vi "Current_Setting_1_7_26_TC9_ramp_working.vi"() -> ()   [LabVIEW 2025]
uses:
  <vilib>/addons/zeromq/socket_type.ctl
  <vilib>/DAQmx/write.llb/DAQmx Write (Analog DBL 1Chan 1Samp).vi
  <vilib>/DAQmx/read.llb/DAQmx Read (Analog DBL 1Chan 1Samp).vi
  <vilib>/DAQmx/read.llb/DAQmx Read (Analog 1D DBL NChan 1Samp).vi
  <vilib>/DAQmx/create/channels.llb/DAQmx Create Channel (AI-Voltage-Basic).vi
  Trimming_Coil_Command.vi
  Trimming_Coil_Monitor.vi
  <vilib>/Waveform/DWDTOps.llb/DWDT Digital to Boolean Array.vi
  GV_TC1.vi
  <vilib>/DAQmx/miscellaneous.llb/DAQmx Fill In Error Info.vi
  <vilib>/DAQmx/create/channels.llb/DAQmx Create Channel (AO-Voltage-Basic).vi
  <vilib>/addons/zeromq/zmq_socket.lvclass
  <vilib>/addons/zeromq/zmq_context.lvclass
  <vilib>/addons/zeromq/zeromq.lvlib
  <resource>/objmgr/daqmx.rc
panel:
  out "Numeric":dbl
  in  "TC9_Set_Point":dbl
  in  "stop":bool
  out "TC1_Command":dbl
  out "Waveform Chart":dbl(graph)
  out "Sign*10":dbl
  in  "Error_TC9":dbl
  in  "Inc/Dec":dbl
  in  "RF":tag
  in  "Others":tag
  out "error out":errorcluster
  out "double precision float":dbl
  out "Source 1":dbl
  out "Source 2":dbl
  out "Source 3":dbl
  out "Source 4":dbl
  out "Source 5":dbl
  out "Source 6":dbl
  out "Source 7":dbl
  out "Source 8":dbl
  out "Source 9":dbl
  out "Source 10":dbl
  out "Source 11":dbl
  out "Source 12":dbl
  out "Source 13":dbl
  out "Source 14":dbl
  out "value":dbl[](array[numeric])
  out "subarray":dbl[](array[numeric])
  out "Boolean array":bool[](array[boolean])
  out "TC 1":dbl
  out "TC 2":dbl
  out "TC 3":dbl
  out "TC 4":dbl
  out "TC 5":dbl
  out "TC 6":dbl
  out "TC 7":dbl
  out "TC 8":dbl
  out "going to Device 9":dbl
  out "going to Device 10":dbl
  out "going to Device 11":dbl
  out "going to Device 12":dbl
  out "going to Device 13":dbl
  out "going to Device 14":dbl
  in  "Numerator":dbl
  in  "Denominator":dbl
  in  "Inc/Dec 2":dbl
  in  "Error_Stop":dbl
  in  "Boolean":bool
  out "Array":dbl[](array[numeric])
  out "max value":i16
  out "Array[0]":dbl
  out "Array 2":dbl[](array[numeric])
  in  "TP1":dbl
  in  "TP2":dbl
  in  "RF 2":dbl
  in  "Beam":dbl
  in  "Boolean 2":bool
  in  "Boolean 3":bool
  out "[0]":bool
  out "[1]":bool
  out "[2]":bool
  out "[3]":bool
  out "others":dbl[](array[numeric]) format="%0.2f"
  out "appended array":dbl[](array[numeric])
  out "x/y":dbl
  # "Beam I"
  # "ESD KV"
  # "ARC V"
  # "Filament C"
  # "Inside Iron"
  # "Outside Iron"
  # "ARC C"
  # "ESD mA"
  # "TC1"
  # "TC2"
  # "TC4"
  # "TC5"
  # "TC6"
  # "TC7"
  # "TC10"
  # "TC9"
  # "TP2"
  # "TP1"
  # "Filament V"
  # "Centering Beam"
  # "TC 12"
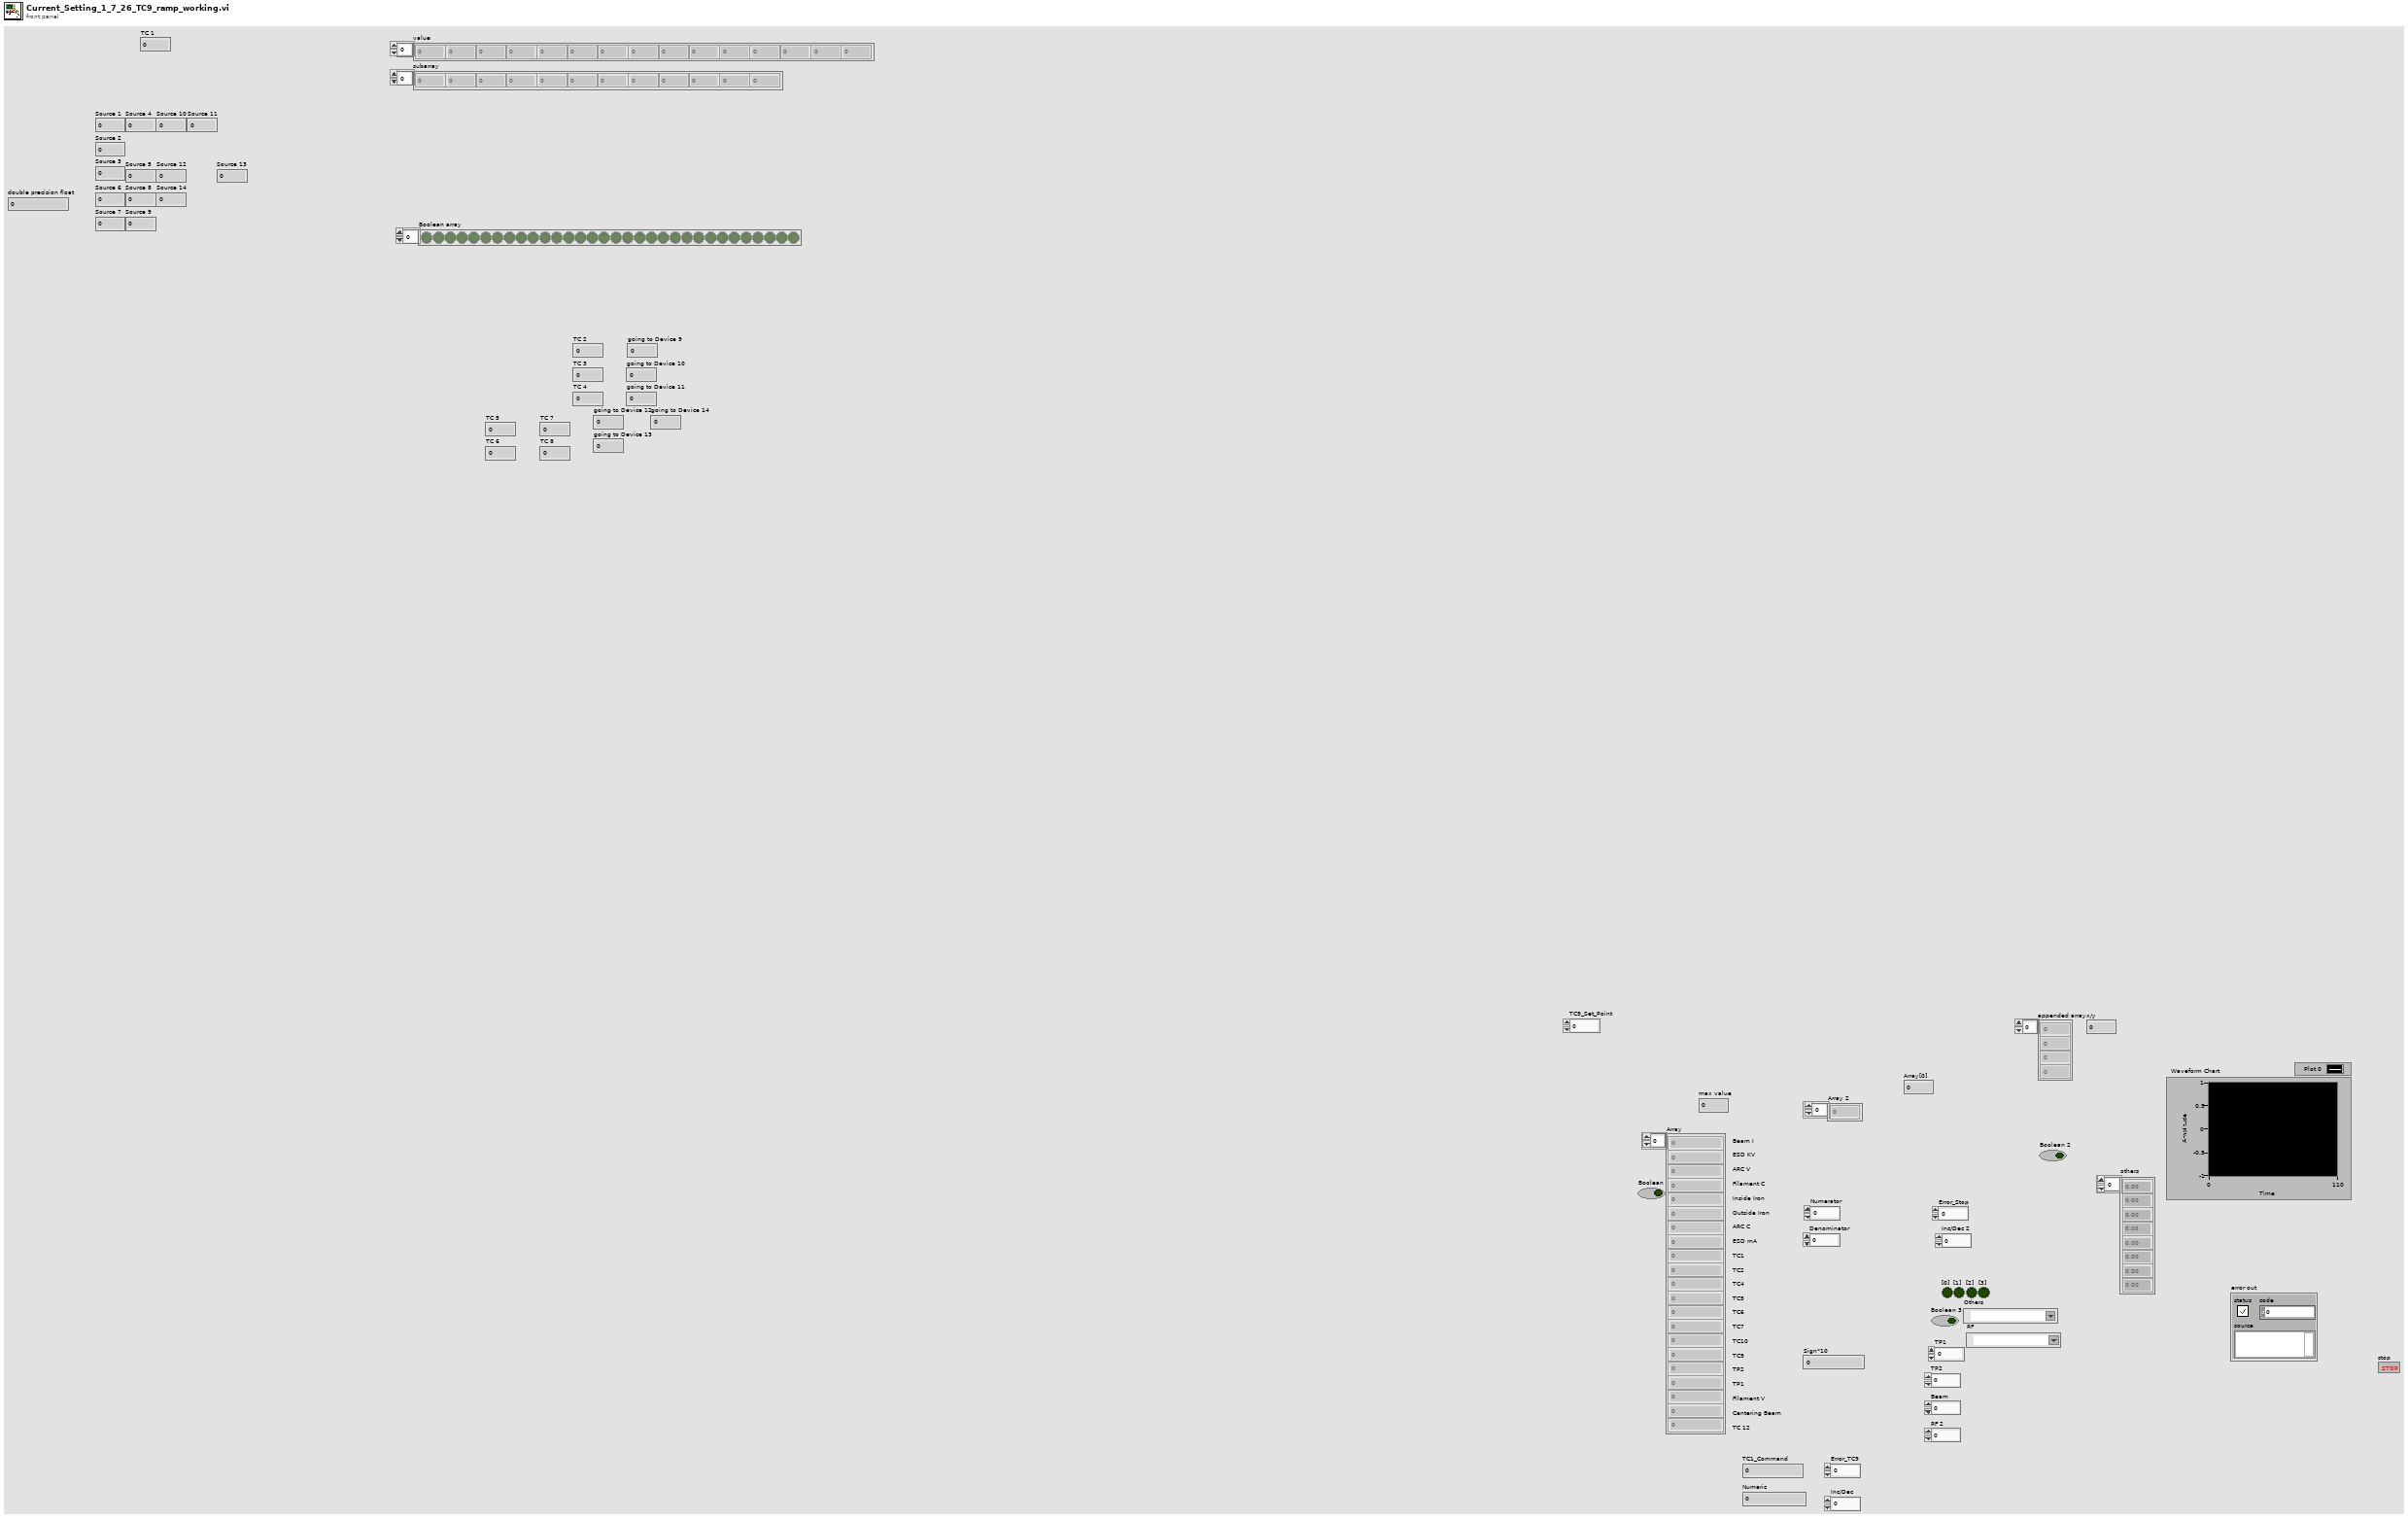
[diagram p1: front panel]
types:
  T1 = typedef "zeromq.lvlib/socket_type.ctl" = enum8{"ZMQ_PAIR", "ZMQ_PUB", "ZMQ_SUB", "ZMQ_REQ", "ZMQ_REP", "ZMQ_DEALER", "ZMQ_ROUTER", "ZMQ_PULL", "ZMQ_PUSH", "ZMQ_XPUB", "ZMQ_XSUB", "ZMQ_STREAM", "ZMQ_SERVER", "ZMQ_CLIENT", "ZMQ_RADIO", "ZMQ_DISH", "ZMQ_GATHER", "ZMQ_SCATTER", "ZMQ_DGRAM"}
  T2 = enum16{"big-endian, network order", "native, host order", "little-endian"}
  T3 = cluster{"TC1_Set_Point":dbl, "TC2_Set_Point":dbl, "TC3_Set_Point":dbl, "TC4_Set_Point":dbl, "TC5_Set_Point":dbl, "TC6_Set_Point":dbl, "TC7_Set_Point":dbl, "TC8_Set_Point":dbl, "TC9_Set_Point":dbl, "TC10_Set_Point":dbl, "TC11_Set_Point":dbl, "TC12_Set_Point":dbl}
  T4 = cluster{"[0]":bool, "[1]":bool, "[2]":bool, "[3]":bool, "[4]":bool, "[5]":bool, "[6]":bool, "[7]":bool, "[8]":bool}
  T5 = cluster{"[0]":dbl, "[1]":dbl, "[2]":dbl, "[3]":dbl, "[4]":dbl, "[5]":dbl, "[6]":dbl, "[7]":dbl}
  T6 = cluster{"Array[0]":dbl, "Array[1]":dbl, "Array[2]":dbl, "Array[3]":dbl, "Array[4]":dbl, "Array[5]":dbl, "Array[6]":dbl, "Array[7]":dbl}
  T7 = cluster{"[0]":digitalwaveform, "[1]":digitalwaveform, "[2]":digitalwaveform, "[3]":digitalwaveform, "[4]":digitalwaveform, "[5]":digitalwaveform, "[6]":digitalwaveform, "[7]":digitalwaveform, "[8]":digitalwaveform}
  T8 = cluster{"TC1_Readback":dbl, "TC2_Readback":dbl, "TC3_Readback":dbl, "TC4_Readback":dbl, "TC5_Readback":dbl, "TC6_Readback":dbl, "TC7_Readback":dbl, "TC8_Readback":dbl, "TC9_Readback":dbl, "TC10_Readback":dbl, "TC11_Readback":dbl, "TC12_Readback":dbl}
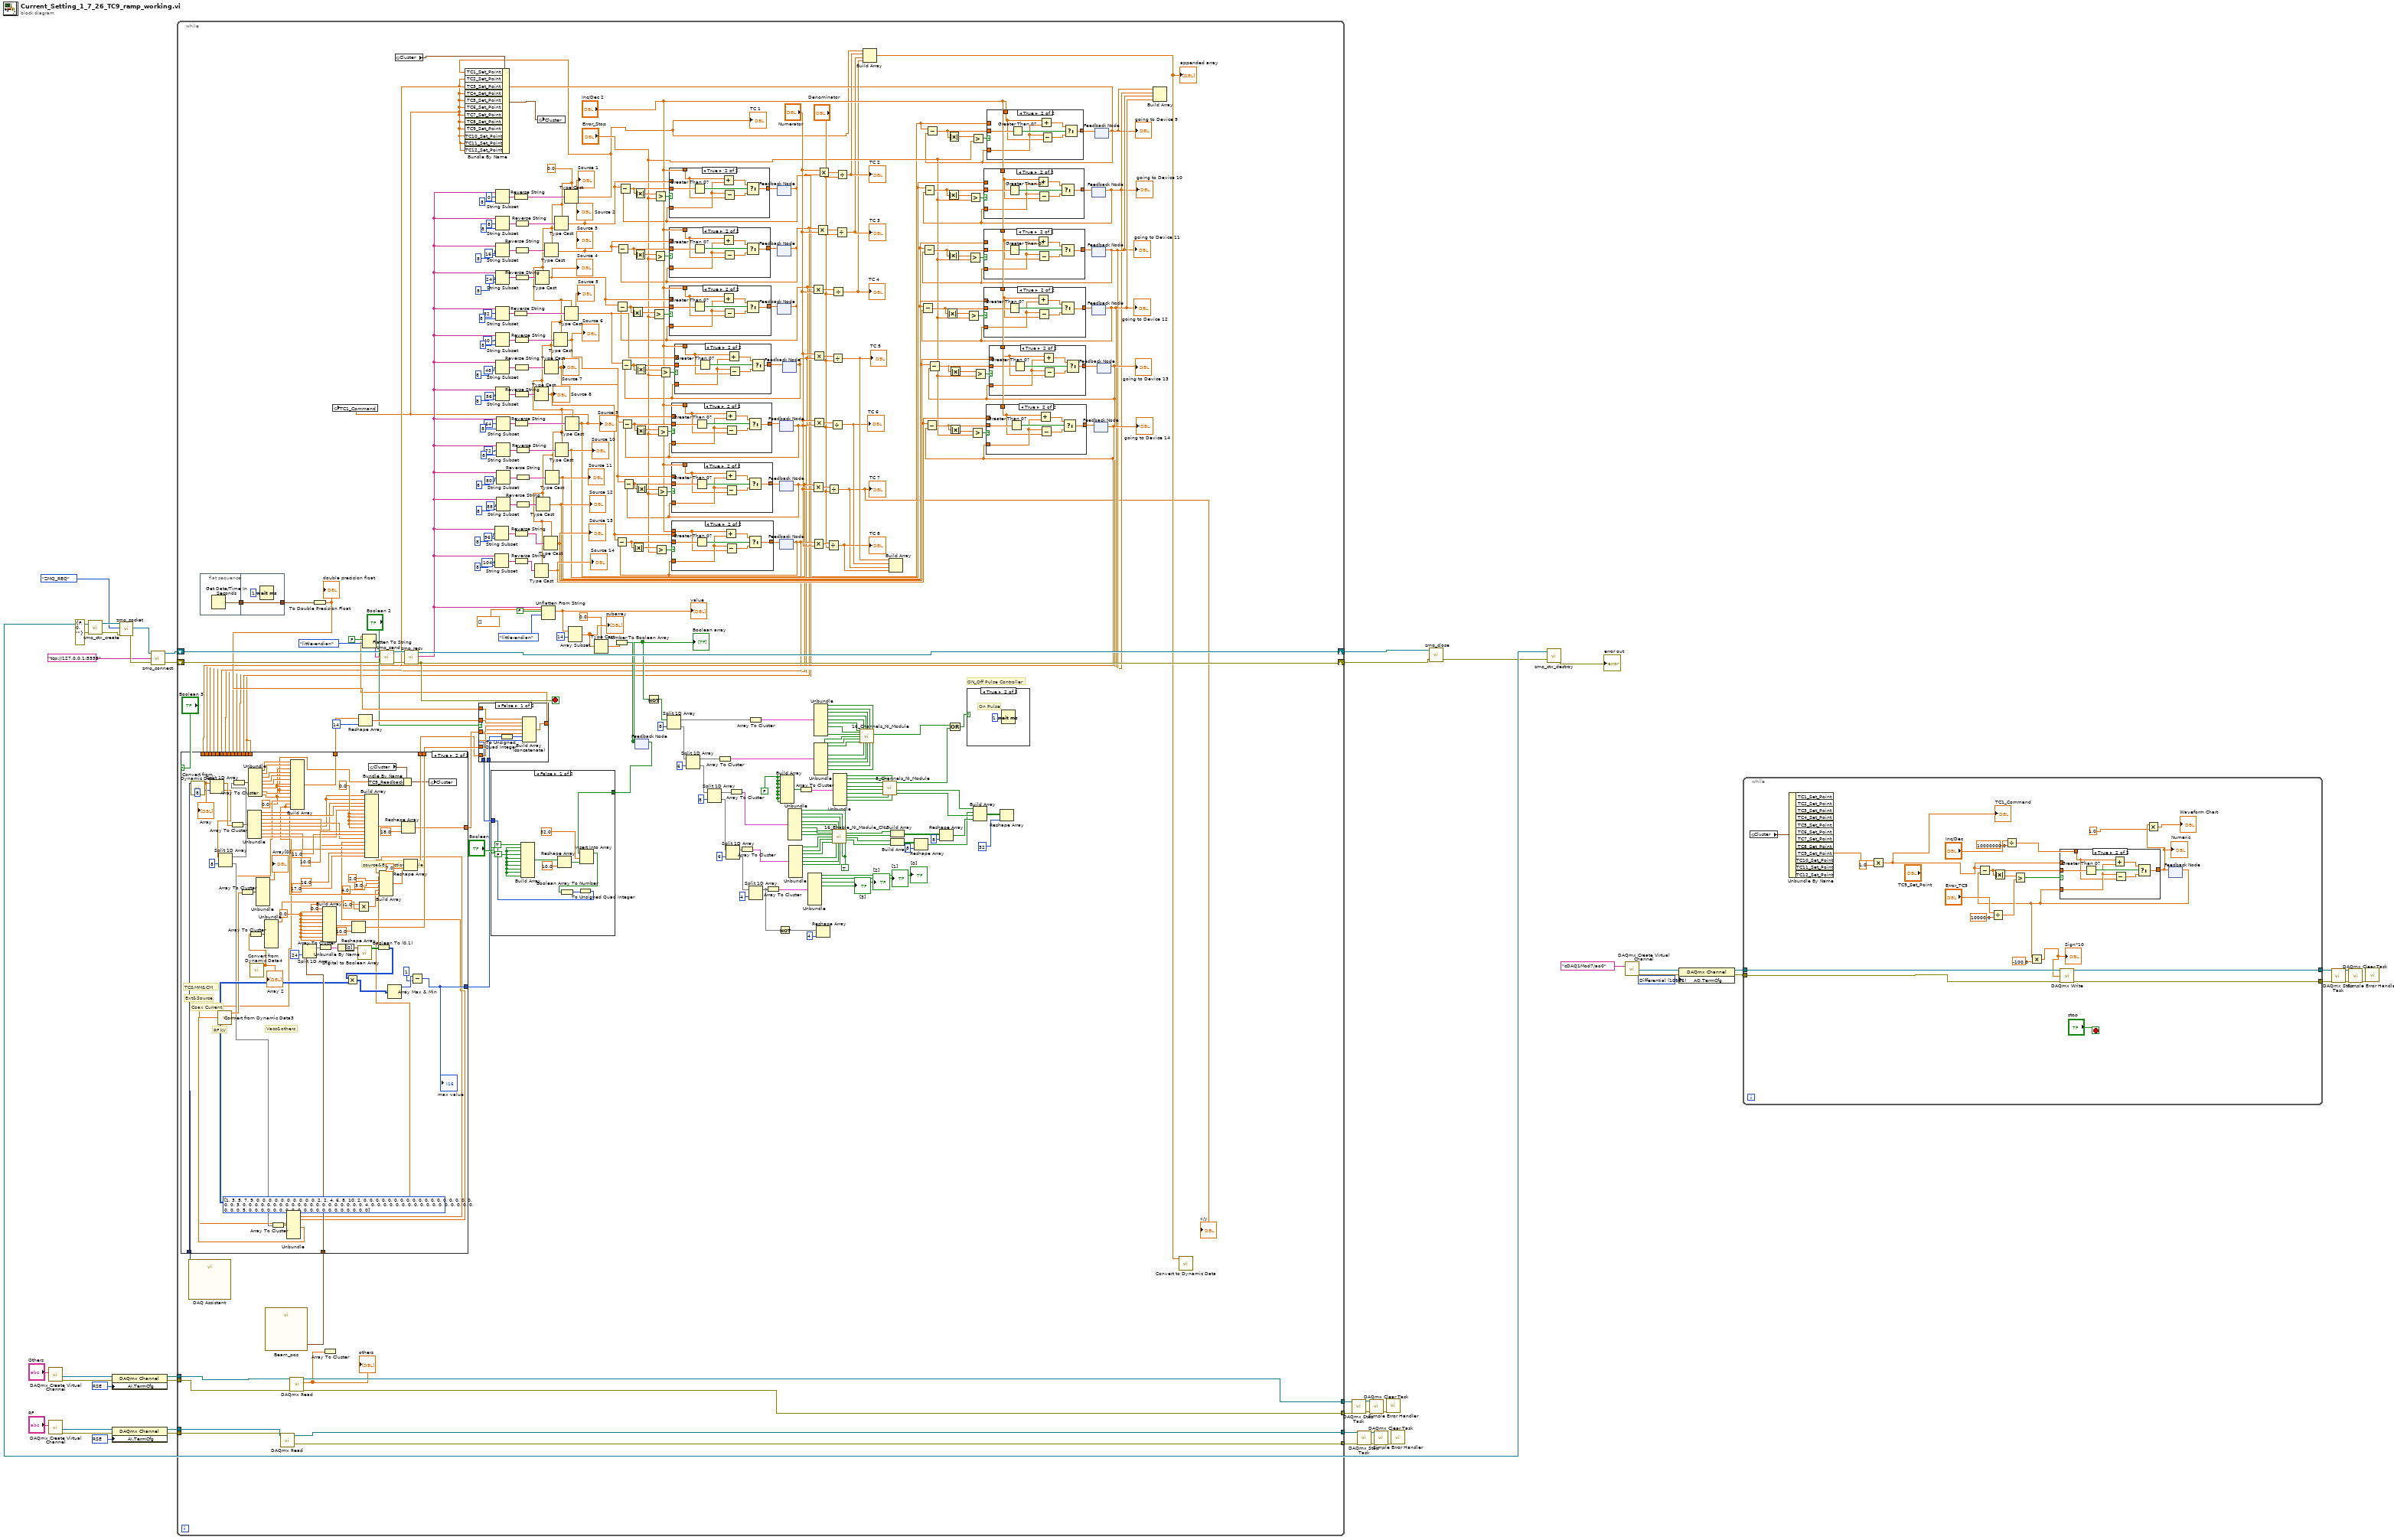
[diagram p0: block diagram]
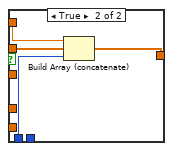
[diagram p3: hidden frame]
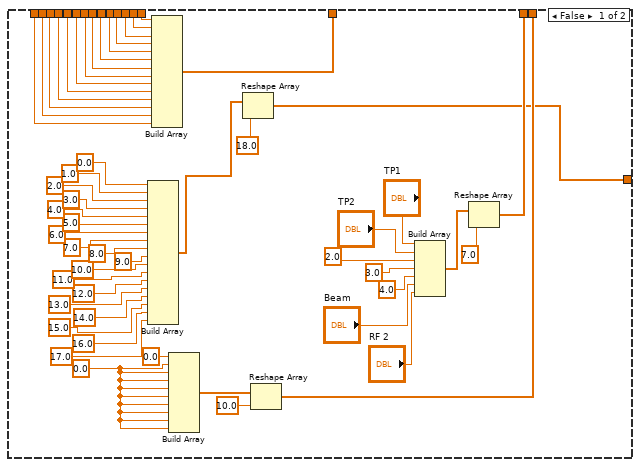
[diagram p4: hidden frame]
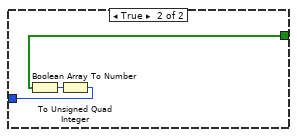
[diagram p5: hidden frame]
diagram:
  w8 = 10106 items=["RSE"=10083, "Differential"=10106, "Pseudodifferential"=12529] ("AO.TermCfg")
  w20 = 10083 items=["RSE"=10083, "Differential"=10106, "Pseudodifferential"=12529] ("AO.TermCfg")
  w31 = 10083 items=["RSE"=10083, "Differential"=10106, "Pseudodifferential"=12529] ("AO.TermCfg")
  n1 = call-poly <vilib>:"DAQmx Create Virtual Channel.vi"("physical channels"="Others") -> ("task out"=w32:refnum<k21>, "error out"=w33:errorcluster)  [unwired: 13 in]
  n2 = call-poly <vilib>:"DAQmx Create Virtual Channel.vi"("physical channels"="RF") -> ("task out"=w21:refnum<k21>, "error out"=w22:errorcluster)  [unwired: 13 in]
  n3 = call <vilib>:"zmq_ctx_create.vi"("error in"=errorcluster {"status"=FALSE, "code"=0, "source"=""}) -> ("error out"=w45:errorcluster, "context out"=w46:refnum<class "zmq_context.lvclass">)  [unwired: 3 in]
  n4 = property class="DAQmx Channel"(reference=w32, error in=w33, "AI.TermCfg"=w31) -> (reference out=w26:refnum<k21>, error out=w25:errorcluster)
  n5 = property class="DAQmx Channel"(reference=w21, error in=w22, "AI.TermCfg"=w20) -> (reference out=w18:refnum<k21>, error out=w17:errorcluster)
  n6 = call <vilib>:"zmq_socket.vi"("error in"=w45, "socket type"=socket_type."ZMQ_REQ", "context in"=w46) -> ("error out"=w43:errorcluster, "socket out"=w44:refnum<class "zmq_socket.lvclass">, "context out"=w38:refnum<class "zmq_context.lvclass">)  [unwired: 2 in]
  n7 = call <vilib>:"zmq_connect.vi"("error in"=w43, "endpoint"="tcp://127.0.0.1:5555", "socket in"=w44) -> ("error out"=w39:errorcluster, "socket out"=w40:refnum<class "zmq_socket.lvclass">)  [unwired: 1 in]
  n8 = while {
    shift-right: [w225] -> w35
    shift-left: w40 -> [w335]
    shift-right: [w224] -> w36
    shift-left: w39 -> [w334]
    tunnel: w26 -> [w82]
    tunnel: w25 -> [w81]
    tunnel: [w80] -> w24
    tunnel: [w79] -> w23
    tunnel: w18 -> [w78]
    tunnel: w17 -> [w77]
    tunnel: [w76] -> w13
    tunnel: [w75] -> w12
    stop <- w224 stop-if-true
    w115 = TRUE
    w118 = FALSE
    w52 = 0.0
    # "ON_Off Pulse Controller"
    n9 = call "DAQ Assistant"() -> ("data"=w57:dynamicdata)  [unwired: 16 in, 3 out]
    n10 = flat-sequence {
      tunnel: [w593] -> w330
      tunnel: [w595] -> w331
      tunnel: w330 -> [w595]
      frame #0 {
        n11 = Get Date/Time In Seconds() -> (seconds since 1Jan1904=w593:timestamp)
      }
      frame #1 {
        n12 = Wait (ms)(milliseconds to wait=u32 1) -> ()  [unwired: 1 out]
      }
    }
    n13 = call "Beam_pos"() -> ("data"=w58:digitalwaveform[])  [unwired: 16 in, 3 out]
    n14 = call-poly <vilib>:"DAQmx Read.vi"("task/channels in"=w78, "error in"=w77) -> ("task out"=w76:refnum<k21>, "error out"=w75:errorcluster)  [unwired: 11 in, 1 out]
    n15 = call-poly <vilib>:"DAQmx Read.vi"("task/channels in"=w82, "error in"=w81) -> ("task out"=w79:refnum<k21>, "data"=w74:dbl[], "error out"=w80:errorcluster)  [unwired: 11 in]
    "others" <- w74
    n16 = To Double Precision Float(number=w331) -> (double precision float=w102:dbl)
    "double precision float" <- w102
    n17 = Array To Cluster(array=w74) -> ()  [unwired: 1 out]
    n18 = global read "Trimming_Coil_Command.vi" "Cluster"() -> (w51:T3)
    n19 = feedback #1() -> (w105:bool[])  [unwired: 1 in]
    n20 = case shown="False" "Boolean" {
      tunnel: w105 -> [w480 w486]
      tunnel: [w477 w485] -> w103
      frame False {
        w483 = FALSE
        n21 = Build Array(TRUE, w483, w483, w483, w483, w483, w483, w483, w483, w483) -> (w482:bool[])
        n22 = Reshape Array(w482, 10.0) -> (w475:bool[])
        n23 = Insert Into Array(array=w480, index=32.0, new element=w475) -> (w478:bool[])
        n24 = Boolean Array To Number(Boolean array=w478) -> (number=w479:u32)
        n25 = To Unsigned Quad Integer(1:w479) -> (0:w477:u64)
      }
      frame True {
        n26 = Boolean Array To Number(Boolean array=w486) -> (number=w487:u32)
        n27 = To Unsigned Quad Integer(1:w487) -> (0:w485:u64)
      }
    }
    n28 = feedback #2() -> (w53:dbl)  [unwired: 1 in]
    n29 = feedback #3() -> (w62:dbl)  [unwired: 1 in]
    n30 = feedback #4() -> (w63:dbl)  [unwired: 1 in]
    n31 = feedback #5() -> (w65:dbl)  [unwired: 1 in]
    n32 = feedback #6() -> (w66:dbl)  [unwired: 1 in]
    n33 = feedback #7() -> (w67:dbl)  [unwired: 1 in]
    n34 = Build Array(w118, w118, w118, w118, w118, w118, w118, w118) -> (w116:bool[])
    n35 = feedback #8() -> (w64:dbl)  [unwired: 1 in]
    n36 = Array To Cluster(array=w116) -> (cluster=w117:T4)
    n37 = Multiply(x=w63, y="Numerator") -> (x*y=w219:dbl)
    n38 = Multiply(x=w66, y="Numerator") -> (x*y=w216:dbl)
    n39 = Multiply(x=w67, y="Numerator") -> (x*y=w215:dbl)
    n40 = Multiply(x="Numerator", y=w64) -> (x*y=w218:dbl)
    n41 = Multiply(x="Numerator", y=w65) -> (x*y=w217:dbl)
    n42 = Multiply(x=w62, y="Numerator") -> (x*y=w220:dbl)
    n43 = Multiply(x="Numerator", y=w53) -> (x*y=w221:dbl)
    n44 = Divide(x=w215, y="Denominator") -> (x/y=w106:dbl)
    "TC 8" <- w106
    n45 = Divide(x=w216, y="Denominator") -> (x/y=w54:dbl)
    "TC 7" <- w54
    "x/y" <- w54
    n46 = Divide(x=w217, y="Denominator") -> (x/y=w107:dbl)
    "TC 6" <- w107
    n47 = Divide(x=w218, y="Denominator") -> (x/y=w108:dbl)
    "TC 5" <- w108
    n48 = Divide(x=w219, y="Denominator") -> (x/y=w109:dbl)
    "TC 4" <- w109
    n49 = Unbundle(w117) -> ("[0]"=w152:bool, "[1]"=w151:bool, "[2]"=w150:bool, "[3]"=w149:bool, "[4]"=w148:bool, "[5]"=w147:bool, "[6]"=w146:bool, "[7]"=w145:bool)  [unwired: 1 out]
    n50 = Divide(x=w220, y="Denominator") -> (x/y=w110:dbl)
    "TC 3" <- w110
    n51 = Divide(x=w221, y="Denominator") -> (x/y=w111:dbl)
    "TC 2" <- w111
    n52 = call "8_Channels_NI_Module.vi"("Trigger 8"=w145, "Trigger"=w152, "Trigger 7"=w146, "Trigger 2"=w151, "Trigger 6"=w147, "Trigger 5"=w148, "Trigger 4"=w149, "Trigger 3"=w150) -> ("Off Array"=w143:bool[], "On Array"=w144:bool[], "Timing"=w114:bool)  [unwired: 1 in]
    n53 = Build Array(w108, w107, w54, w106) -> ()  [unwired: 1 out]
    n54 = feedback #9() -> (w69:dbl)  [unwired: 1 in]
    "going to Device 10" <- w69
    n55 = feedback #10() -> (w70:dbl)  [unwired: 1 in]
    "going to Device 11" <- w70
    n56 = feedback #11() -> (w71:dbl)  [unwired: 1 in]
    "going to Device 12" <- w71
    n57 = feedback #12() -> (w73:dbl)  [unwired: 1 in]
    "going to Device 14" <- w73
    n58 = feedback #13() -> (w68:dbl)  [unwired: 1 in]
    "going to Device 9" <- w68
    n59 = feedback #14() -> (w72:dbl)  [unwired: 1 in]
    "going to Device 13" <- w72
    n60 = case shown="True" "Boolean 3" {
      tunnel: [w374 w463] -> w97
      tunnel: [w368 w458] -> w96
      tunnel: [w371 w461] -> w95
      tunnel: w57 -> [_ w455]
      tunnel: w73 -> [w363 _]
      tunnel: w72 -> [w362 _]
      tunnel: w71 -> [w361 _]
      tunnel: w70 -> [w360 _]
      tunnel: w69 -> [w359 _]
      tunnel: w68 -> [w358 _]
      tunnel: w67 -> [w357 _]
      tunnel: w66 -> [w356 _]
      tunnel: w65 -> [w355 _]
      tunnel: w64 -> [w354 _]
      tunnel: w63 -> [w353 _]
      tunnel: w62 -> [w352 _]
      tunnel: w53 -> [w351 _]
      tunnel: w53 -> [w350 _]
      tunnel: [w349 w456] -> w60
      tunnel: w58 -> [_ w438]
      tunnel: [_ w426] -> w56
      frame False {
        w375 = 0.0 ("element")
        n61 = Build Array(0.0, 1.0, 2.0, 3.0, 4.0, 5.0, 6.0, 7.0, 8.0, 9.0, 10.0, 11.0, 12.0, 13.0, 14.0, 15.0, 16.0, 17.0) -> (w369:dbl[])
        n62 = Build Array(w350, w351, w352, w353, w354, w355, w356, w357, w358, w359, w360, w361, w362, w363) -> (w349:dbl[])
        n63 = Build Array(0.0 ("element"), w375, w375, w375, w375, w375, w375, w375, w375, w375) -> (w378:dbl[])
        n64 = Reshape Array(w369, 18.0) -> (w368:dbl[])
        n65 = Reshape Array(w378, 10.0) -> (w374:dbl[])
        n66 = Build Array("TP1", "TP2", 2.0, 3.0, 4.0, "Beam", "RF 2") -> (w372:dbl[])
        n67 = Reshape Array(w372, 7.0) -> (w371:dbl[])
      }
      frame True {
        w405 = 0.0
        w457 = 0.0
        w465 = 0.0 ("element")
        # "RF kV"
        # "Coax Current"
        # "Vacs&others"
        # "Ext&Source"
        # "TC&MM&CM"
        # "source&Extraction&angle"
        n68 = call "Convert from Dynamic Data"("Dynamic Data Type"=w455) -> ("Array"=w446:dbl[])  [unwired: 3 in]
        "Array" <- w446
        n69 = Split 1D Array(array=w446, index=8) -> (first subarray=w409:dbl[], second subarray=w408:dbl[])
        n70 = call "Convert from Dynamic Data3"() -> ("Array"=w428:dbl[])  [unwired: 4 in]
        n71 = Split 1D Array(array=w408, index=8) -> (first subarray=w407:dbl[], second subarray=w416:dbl[])
        n72 = Array To Cluster(array=w409) -> (cluster=w444:T5)
        n73 = Array To Cluster(array=w407) -> (cluster=w447:T5)
        n74 = Array To Cluster(array=w428) -> (cluster=w429:T6)
        n75 = Unbundle(w444) -> ("[0]"=w430:dbl, "[1]"=w443:dbl, "[2]"=w441:dbl, "[3]"=w440:dbl, "[4]"=w410:dbl, "[5]"=w411:dbl, "[6]"=w413:dbl, "[7]"=w442:dbl)
        n76 = Unbundle(w447) -> ("[0]"=w403:dbl, "[1]"=w454:dbl, "[2]"=w453:dbl, "[3]"=w452:dbl, "[4]"=w451:dbl, "[5]"=w450:dbl, "[6]"=w449:dbl, "[7]"=w400:dbl)
        n77 = call "Convert from Dynamic Data4"() -> ("Array"=w421:dbl[])  [unwired: 4 in]
        "Array 2" <- w421
        n78 = Array To Cluster(array=w421) -> (cluster=w422:T6)
        n79 = Unbundle(w429) -> ("Array[0]"=→"Array[0]":dbl)  [unwired: 7 out]
        n80 = Unbundle(w422) -> ("Array[0]"=w420:dbl)  [unwired: 7 out]
        n81 = Array To Cluster(array=w416) -> (cluster=w418:T5)
        n82 = Unbundle(w418) -> ("[0]"=w415:dbl, "[1]"=w414:dbl, "[2]"=w412:dbl, "[3]"=w404:dbl, "[4]"=w406:dbl)  [unwired: 3 out]
        n83 = Build Array(w403, w454, w405, w453, w452, w451, w450, w405, w400, w449, w405, w406, w404, w404) -> (w456:dbl[])
        n84 = Split 1D Array(array=w438, index=24) -> (first subarray=w435:digitalwaveform[])  [unwired: 1 out]
        n85 = Array To Cluster(array=w435) -> (cluster=w437:T7)
        n86 = Build Array(0.0 ("element"), w465, w465, w465, w465, w465, w465, w465, w465, w465) -> (w468:dbl[])
        n87 = Unbundle By Name(w437) -> ("[0]"=w436:digitalwaveform)
        n88 = Reshape Array(w468, 10.0) -> (w463:dbl[])
        n89 = Multiply(x=-1.0, y=w420) -> (x*y=w423:dbl)
        n90 = call-poly <vilib>:"Digital to Boolean Array.vi"("digital waveform"=w436) -> ("boolean array"=w434:bool[][])  [unwired: 9 in, 1 out]
        n91 = Build Array(w410, w410, w411, w443, w442, w457, w457, w457, w457, w457, 10.0, 11.0, w440, w412, w441, w413, 16.0, 17.0) -> (w459:dbl[])
        n92 = global read "Trimming_Coil_Monitor.vi" "Cluster"() -> (w402:T8)
        n93 = Bundle By Name(cluster=w402, "TC9_Readback"=w400) -> (w401:T8)
        n94 = Boolean To (0,1)(Boolean=w434) -> (0, 1=w433:i16[][])
        n95 = Multiply(x=w433, y=i16[][] [[1, 3, 5, 7, 9, 0, 0, 0, 0, 0, 0, 0, 0, 0, 0, 2, 2, 4, 6, 8, 10], [2, 0, 0, 0, 0, 0, 0, 0, 0, 0, 0, 0, 0, 0, 0, 0, 0, 0, 0, 0, 0], [3, 0, 0, 0, 0, 0, 0, 0, 0, 0, 0, 0, 0, 0, 0, 0, 0, 0, 0, 0, 0], [4, 0, 0, 0, 0, 0, 0, 0, 0, 0, 0, 0, 0, 0, 0, 0, 0, 0, 0, 0, 0], [5, 0, 0, 0, 0, 0, 0, 0, 0, 0, 0, 0, 0, 0, 0, 0, 0, 0, 0, 0, 0]]) -> (x*y=w431:i16[][])
        n96 = Build Array(w414, w415, 2.0, 3.0, 4.0, w423, w430) -> (w462:dbl[])
        n97 = Array Max & Min(array=w431) -> (max value=w425:i16)  [unwired: 3 out]
        n98 = Reshape Array(w459, 18.0) -> (w458:dbl[])
        n99 = Reshape Array(w462, 7.0) -> (w461:dbl[])
        n100 = Subtract(x=w425, y=i16 1 ("x")) -> (x-y=w426:i16)
        "max value" <- w426
        n101 = global write "Trimming_Coil_Monitor.vi" "Cluster"(w401) -> ()
      }
    }
    n102 = Reshape Array(w60, 14 ("dimension size")) -> (w101:dbl[])
    n103 = case shown="False" "Boolean 2" {
      tunnel: w103 -> [w338 w348]
      tunnel: w102 -> [w344 w347]
      tunnel: w101 -> [w343 w346]
      tunnel: [w342 w345] -> w100
      tunnel: w97 -> [w340 _]
      tunnel: w96 -> [w341 _]
      tunnel: w95 -> [w339 _]
      tunnel: w56 -> [w336 _]
      frame False {
        n104 = To Unsigned Quad Integer(1:w336) -> (0:w337:u64)
        n105 = Build Array (concatenate)(w344, w343, w341, w340, w339, w337, w338) -> (w342:dbl[])
      }
      frame True {
        n106 = Build Array (concatenate)(w347, w346, w348) -> (w345:dbl[])
      }
    }
    n107 = Flatten To String(anything=w100, prepend array or string size? (T)=FALSE, byte order (0:big-endian, network order)=T2."little-endian") -> (data string=w223:string)  [unwired: 1 in, 2 out]
    n108 = call <vilib>:"zmq_send.vi"("error in"=w334, "data"=w223, "socket in"=w335) -> ("error out"=w332:errorcluster, "socket out"=w333:refnum<class "zmq_socket.lvclass">)  [unwired: 4 in]
    n109 = call <vilib>:"zmq_recv.vi"("error in"=w332, "socket in"=w333) -> ("error out"=w224:errorcluster, "data"=w222:string, "socket out"=w225:refnum<class "zmq_socket.lvclass">)  [unwired: 3 in, 2 out]
    n110 = String Subset(string=w222, offset (0)=96, length (rest)=8 ("length (rest)")) -> (substring=w275:string)
    n111 = String Subset(string=w222, offset (0)=104, length (rest)=8 ("length (rest)")) -> (substring=w273:string)
    n112 = String Subset(string=w222, offset (0)=32, length (rest)=8 ("length (rest)")) -> (substring=w307:string)
    n113 = String Subset(string=w222, offset (0)=40, length (rest)=8 ("length (rest)")) -> (substring=w305:string)
    n114 = String Subset(string=w222, offset (0)=48, length (rest)=8 ("length (rest)")) -> (substring=w299:string)
    n115 = String Subset(string=w222, offset (0)=56, length (rest)=8 ("length (rest)")) -> (substring=w297:string)
    n116 = String Subset(string=w222, offset (0)=0, length (rest)=8 ("length (rest)")) -> (substring=w323:string)
    n117 = String Subset(string=w222, offset (0)=8, length (rest)=8 ("length (rest)")) -> (substring=w321:string)
    n118 = String Subset(string=w222, offset (0)=16, length (rest)=8 ("length (rest)")) -> (substring=w315:string)
    n119 = String Subset(string=w222, offset (0)=24, length (rest)=8 ("length (rest)")) -> (substring=w313:string)
    n120 = String Subset(string=w222, offset (0)=64, length (rest)=8 ("length (rest)")) -> (substring=w291:string)
    n121 = String Subset(string=w222, offset (0)=72, length (rest)=8 ("length (rest)")) -> (substring=w289:string)
    n122 = String Subset(string=w222, offset (0)=80, length (rest)=8 ("length (rest)")) -> (substring=w283:string)
    n123 = String Subset(string=w222, offset (0)=88, length (rest)=8 ("length (rest)")) -> (substring=w281:string)
    n124 = Reverse String(1:w307) -> (0:w306:string)
    n125 = Reverse String(1:w323) -> (0:w322:string)
    n126 = Reverse String(1:w291) -> (0:w290:string)
    n127 = Reverse String(1:w275) -> (0:w274:string)
    n128 = Reverse String(1:w273) -> (0:w272:string)
    n129 = Reverse String(1:w305) -> (0:w304:string)
    n130 = Reverse String(1:w299) -> (0:w298:string)
    n131 = Reverse String(1:w297) -> (0:w296:string)
    n132 = Reverse String(1:w321) -> (0:w320:string)
    n133 = Reverse String(1:w315) -> (0:w314:string)
    n134 = Reverse String(1:w313) -> (0:w312:string)
    n135 = Reverse String(1:w289) -> (0:w288:string)
    n136 = Reverse String(1:w283) -> (0:w282:string)
    n137 = Reverse String(1:w281) -> (0:w280:string)
    n138 = Type Cast(type=w52, x=w272) -> (*(type *) &x=w230:dbl)
    "Source 14" <- w230
    n139 = Type Cast(type=w52, x=w296) -> (*(type *) &x=w243:dbl)
    "Source 8" <- w243
    n140 = Type Cast(type=w52, x=w312) -> (*(type *) &x=w255:dbl)
    "Source 4" <- w255
    n141 = Type Cast(type=w52, x=w280) -> (*(type *) &x=w228:dbl)
    "Source 12" <- w228
    n142 = Unflatten From String(type=dbl[] [], binary string=w222, data includes array or string size? (T)=FALSE, byte order (0:big-endian, network order)=T2."little-endian") -> (value=w268:dbl[])  [unwired: 1 in, 2 out]
    "value" <- w268
    n143 = Type Cast(type=w52, x=w274) -> (*(type *) &x=w229:dbl)
    "Source 13" <- w229
    n144 = Type Cast(type=w52, x=w298) -> (*(type *) &x=w244:dbl)
    "Source 7" <- w244
    n145 = Type Cast(type=w52, x=w314) -> (*(type *) &x=w256:dbl)
    "Source 3" <- w256
    n146 = Type Cast(type=w52, x=w282) -> (*(type *) &x=w227:dbl)
    "Source 11" <- w227
    n147 = Type Cast(type=w52, x=w304) -> (*(type *) &x=w245:dbl)
    "Source 6" <- w245
    n148 = Type Cast(type=w52, x=w320) -> (*(type *) &x=w257:dbl)
    "Source 2" <- w257
    n149 = Type Cast(type=w52, x=w288) -> (*(type *) &x=w226:dbl)
    "Source 10" <- w226
    n150 = Type Cast(type=w52, x=w306) -> (*(type *) &x=w246:dbl)
    "Source 5" <- w246
    n151 = Type Cast(type=w52, x=w322) -> (*(type *) &x=w49:dbl)
    "Source 1" <- w49
    "TC 1" <- w49
    n152 = Type Cast(type=w52, x=w290) -> (*(type *) &x=w48:dbl)
    "Source 9" <- w48
    n153 = global write "GV_TC1.vi" "TC1_Command"(w48) -> ()
    n154 = Bundle By Name(cluster=w51, "TC1_Set_Point"=w49, "TC2_Set_Point"=w48, "TC3_Set_Point"=w48, "TC4_Set_Point"=w48, "TC5_Set_Point"=w48, "TC6_Set_Point"=w48, "TC7_Set_Point"=w48, "TC8_Set_Point"=w48, "TC9_Set_Point"=w48, "TC10_Set_Point"=w48, "TC11_Set_Point"=w48, "TC12_Set_Point"=w48) -> (w50:T3)
    n155 = global write "Trimming_Coil_Command.vi" "Cluster"(w50) -> ()
    n156 = Array Subset(array=w268, index=14) -> (w266:dbl[])  [unwired: 1 in]
    "subarray" <- w266
    n157 = Type Cast(type=0.0, x=w266) -> (*(type *) &x=w264:dbl)
    n158 = Number To Boolean Array(number=w264) -> (Boolean array=w204:bool[])
    "Boolean array" <- w204
    n159 = Subtract(x=w243, y=w67) -> (x-y=w193:dbl)
    n160 = Subtract(x=w255, y=w63) -> (x-y=w198:dbl)
    n161 = Subtract(x=w256, y=w62) -> (x-y=w199:dbl)
    n162 = Subtract(x=w257, y=w53) -> (x-y=w202:dbl)
    n163 = Subtract(x=w246, y=w64) -> (x-y=w195:dbl)
    n164 = Subtract(x=w245, y=w65) -> (x-y=w190:dbl)
    n165 = Subtract(x=w244, y=w66) -> (x-y=w192:dbl)
    n166 = Absolute Value(x=w198) -> (abs(x)=w197:dbl)
    n167 = Absolute Value(x=w193) -> (abs(x)=w194:dbl)
    n168 = Absolute Value(x=w202) -> (abs(x)=w201:dbl)
    n169 = Absolute Value(x=w199) -> (abs(x)=w200:dbl)
    n170 = Absolute Value(x=w195) -> (abs(x)=w196:dbl)
    n171 = Absolute Value(x=w190) -> (abs(x)=w189:dbl)
    n172 = Absolute Value(x=w192) -> (abs(x)=w191:dbl)
    n173 = feedback-in #1(w204) -> ()
    n174 = Not(x=w204) -> (.not. x?=w203:bool[])
    n175 = Greater?(x=w197, y="Error_Stop") -> (0:w259:bool)
    n176 = Greater?(x=w200, y="Error_Stop") -> (0:w261:bool)
    n177 = Greater?(x=w201, y="Error_Stop") -> (0:w263:bool)
    n178 = Greater?(x=w194, y="Error_Stop") -> (0:w248:bool)
    n179 = Greater?(x=w191, y="Error_Stop") -> (0:w250:bool)
    n180 = Greater?(x=w189, y="Error_Stop") -> (0:w252:bool)
    n181 = Greater?(x=w196, y="Error_Stop") -> (0:w254:bool)
    n182 = Split 1D Array(array=w203, index=8) -> (first subarray=w213:bool[], second subarray=w212:bool[])
    n183 = case shown="True" w263 {
      tunnel: w202 -> [_ w592]
      tunnel: w53 -> [_ w590]
      tunnel: [w585 w587] -> w262
      tunnel: w257 -> [w585 _]
      tunnel: "Inc/Dec 2" -> [_ w586]
      frame False {
      }
      frame True {
        n184 = Greater Than 0?(x=w592) -> (x > 0?=w591:bool)
        n185 = Add(x=w586, y=w590) -> (x+y=w588:dbl)
        n186 = Subtract(x=w590, y=w586) -> (x-y=w589:dbl)
        n187 = Select(t=w588, s=w591, f=w589) -> (s? t:f=w587:dbl)
      }
    }
    n188 = case shown="True" w261 {
      tunnel: w199 -> [_ w584]
      tunnel: w62 -> [_ w582]
      tunnel: [w577 w579] -> w260
      tunnel: w256 -> [w577 _]
      tunnel: "Inc/Dec 2" -> [_ w578]
      frame False {
      }
      frame True {
        n189 = Greater Than 0?(x=w584) -> (x > 0?=w583:bool)
        n190 = Add(x=w578, y=w582) -> (x+y=w580:dbl)
        n191 = Subtract(x=w582, y=w578) -> (x-y=w581:dbl)
        n192 = Select(t=w580, s=w583, f=w581) -> (s? t:f=w579:dbl)
      }
    }
    n193 = case shown="True" w259 {
      tunnel: w198 -> [_ w576]
      tunnel: w63 -> [_ w574]
      tunnel: [w569 w571] -> w258
      tunnel: w255 -> [w569 _]
      tunnel: "Inc/Dec 2" -> [_ w570]
      frame False {
      }
      frame True {
        n194 = Greater Than 0?(x=w576) -> (x > 0?=w575:bool)
        n195 = Add(x=w570, y=w574) -> (x+y=w572:dbl)
        n196 = Subtract(x=w574, y=w570) -> (x-y=w573:dbl)
        n197 = Select(t=w572, s=w575, f=w573) -> (s? t:f=w571:dbl)
      }
    }
    n198 = case shown="True" w252 {
      tunnel: w190 -> [_ w560]
      tunnel: w65 -> [_ w558]
      tunnel: [w553 w555] -> w251
      tunnel: w245 -> [w553 _]
      tunnel: "Inc/Dec 2" -> [_ w554]
      frame False {
      }
      frame True {
        n199 = Greater Than 0?(x=w560) -> (x > 0?=w559:bool)
        n200 = Add(x=w554, y=w558) -> (x+y=w556:dbl)
        n201 = Subtract(x=w558, y=w554) -> (x-y=w557:dbl)
        n202 = Select(t=w556, s=w559, f=w557) -> (s? t:f=w555:dbl)
      }
    }
    n203 = case shown="True" w250 {
      tunnel: w192 -> [_ w552]
      tunnel: w66 -> [_ w550]
      tunnel: [w545 w547] -> w249
      tunnel: w244 -> [w545 _]
      tunnel: "Inc/Dec 2" -> [_ w546]
      frame False {
      }
      frame True {
        n204 = Greater Than 0?(x=w552) -> (x > 0?=w551:bool)
        n205 = Add(x=w546, y=w550) -> (x+y=w548:dbl)
        n206 = Subtract(x=w550, y=w546) -> (x-y=w549:dbl)
        n207 = Select(t=w548, s=w551, f=w549) -> (s? t:f=w547:dbl)
      }
    }
    n208 = case shown="True" w248 {
      tunnel: w193 -> [_ w544]
      tunnel: w67 -> [_ w542]
      tunnel: [w537 w539] -> w247
      tunnel: w243 -> [w537 _]
      tunnel: "Inc/Dec 2" -> [_ w538]
      frame False {
      }
      frame True {
        n209 = Greater Than 0?(x=w544) -> (x > 0?=w543:bool)
        n210 = Add(x=w538, y=w542) -> (x+y=w540:dbl)
        n211 = Subtract(x=w542, y=w538) -> (x-y=w541:dbl)
        n212 = Select(t=w540, s=w543, f=w541) -> (s? t:f=w539:dbl)
      }
    }
    n213 = case shown="True" w254 {
      tunnel: w195 -> [_ w568]
      tunnel: w64 -> [_ w566]
      tunnel: [w561 w563] -> w253
      tunnel: w246 -> [w561 _]
      tunnel: "Inc/Dec 2" -> [_ w562]
      frame False {
      }
      frame True {
        n214 = Greater Than 0?(x=w568) -> (x > 0?=w567:bool)
        n215 = Add(x=w562, y=w566) -> (x+y=w564:dbl)
        n216 = Subtract(x=w566, y=w562) -> (x-y=w565:dbl)
        n217 = Select(t=w564, s=w567, f=w565) -> (s? t:f=w563:dbl)
      }
    }
    n218 = Split 1D Array(array=w212, index=6) -> (first subarray=w210:bool[], second subarray=w208:bool[])
    n219 = Split 1D Array(array=w208, index=8) -> (first subarray=w207:bool[], second subarray=w205:bool[])
    n220 = Array To Cluster(array=w210) -> (cluster=w153:T4)
    n221 = Split 1D Array(array=w205, index=6) -> (first subarray=w206:bool[], second subarray=w92:bool[])
    n222 = Array To Cluster(array=w207) -> (cluster=w112:T4)
    n223 = Array To Cluster(array=w206) -> (cluster=w113:T4)
    n224 = Array To Cluster(array=w213) -> (cluster=w156:T4)
    n225 = Split 1D Array(array=w92, index=4) -> (first subarray=w84:bool[])  [unwired: 1 out]
    n226 = Array To Cluster(array=w84) -> (cluster=w91:T4)
    n227 = feedback-in #2(w262) -> ()
    n228 = feedback-in #3(w260) -> ()
    n229 = feedback-in #4(w258) -> ()
    n230 = Not(x=w84) -> (.not. x?=w83:bool[])
    n231 = feedback-in #5(w251) -> ()
    n232 = feedback-in #6(w249) -> ()
    n233 = feedback-in #7(w247) -> ()
    n234 = feedback-in #8(w253) -> ()
    n235 = Unbundle(w112) -> ("[0]"=w142:bool, "[1]"=w141:bool, "[2]"=w140:bool, "[3]"=w139:bool, "[4]"=w138:bool, "[5]"=w137:bool, "[6]"=w136:bool, "[7]"=w135:bool)  [unwired: 1 out]
    n236 = Unbundle(w113) -> ("[0]"=w130:bool, "[1]"=w129:bool, "[2]"=w128:bool, "[3]"=w127:bool, "[4]"=w94:bool, "[5]"=w93:bool)  [unwired: 3 out]
    n237 = Unbundle(w91) -> ("[0]"=→"[0]":bool, "[1]"=→"[1]":bool, "[2]"=→"[2]":bool, "[3]"=→"[3]":bool)  [unwired: 5 out]
    n238 = Unbundle(w156) -> ("[0]"=w157:bool, "[1]"=w172:bool, "[2]"=w171:bool, "[3]"=w170:bool, "[4]"=w169:bool, "[5]"=w168:bool, "[6]"=w167:bool, "[7]"=w166:bool)  [unwired: 1 out]
    n239 = Unbundle(w153) -> ("[0]"=w165:bool, "[1]"=w164:bool, "[2]"=w163:bool, "[3]"=w162:bool, "[4]"=w161:bool, "[5]"=w160:bool, "[6]"=w159:bool, "[7]"=w158:bool)  [unwired: 1 out]
    n240 = Reshape Array(w83, 4 ("dimension size")) -> ()  [unwired: 1 out]
    n241 = call "16_Enable_NI_Module_CNL.vi"("Enable 6"=w137, "Enable 7"=w136, "Enable 8"=w135, "Enable 9"=w130, "Enable 10"=w129, "Enable 11"=w128, "Enable 5"=w138, "Enable 12"=w127, "Enable 4"=w139, "Enable 13"=w94, "Enable 3"=w140, "Enable 14"=w93, "Enable 2"=w141, "Enable 15"=w115, "Enable 1"=w142, "Enable16"=w115) -> ("9_11_13_15"=w134:bool[], "1_3_5_7"=w133:bool[], "10_12_14_16"=w125:bool[], "2_4_6_8"=w124:bool[])
    n242 = call "16_Channels_NI_Module.vi"("Trigger 6"=w168, "Trigger 7"=w167, "Trigger 8"=w166, "Trigger 9"=w165, "Trigger 10"=w164, "Trigger 11"=w163, "Trigger 5"=w169, "Trigger 12"=w162, "Trigger 4"=w170, "Trigger 13"=w161, "Trigger 3"=w171, "Trigger 14"=w160, "Trigger 2"=w172, "Trigger 15"=w159, "Trigger"=w157, "Trigger 16"=w158) -> ("Timing"=w154:bool)  [unwired: 2 in, 1 out]
    n243 = Build Array(w49, w111, w110, w109) -> (w55:dbl[])
    "appended array" <- w55
    n244 = Build Array(w134, w133) -> (w131:bool[][])
    n245 = Build Array(w125, w124) -> (w123:bool[][])
    n246 = Reshape Array(w123, 8 ("dimension size")) -> (w119:bool[])
    n247 = Subtract(x=w228, y=w71) -> (x-y=w181:dbl)
    n248 = Subtract(x=w227, y=w70) -> (x-y=w183:dbl)
    n249 = Subtract(x=w226, y=w69) -> (x-y=w185:dbl)
    n250 = Subtract(x=w230, y=w73) -> (x-y=w177:dbl)
    n251 = Subtract(x=w48, y=w68) -> (x-y=w187:dbl)
    n252 = Subtract(x=w229, y=w72) -> (x-y=w179:dbl)
    n253 = Reshape Array(w131, 8 ("dimension size")) -> (w120:bool[])
    n254 = Absolute Value(x=w181) -> (abs(x)=w182:dbl)
    n255 = Absolute Value(x=w185) -> (abs(x)=w186:dbl)
    n256 = Absolute Value(x=w183) -> (abs(x)=w184:dbl)
    n257 = Absolute Value(x=w187) -> (abs(x)=w188:dbl)
    n258 = Absolute Value(x=w179) -> (abs(x)=w180:dbl)
    n259 = Absolute Value(x=w177) -> (abs(x)=w178:dbl)
    n260 = Compound Arithmetic op=OR(w154, w114) -> (w155:bool)
    n261 = Greater?(x=w182, y="Error_Stop") -> (0:w236:bool)
    n262 = case shown="True" w155 {
      frame False {
      }
      frame True {
        # "On Pulse"
        n263 = Wait (ms)(milliseconds to wait=u32 1) -> ()  [unwired: 1 out]
      }
    }
    n264 = Greater?(x=w184, y="Error_Stop") -> (0:w238:bool)
    n265 = Greater?(x=w186, y="Error_Stop") -> (0:w240:bool)
    n266 = Greater?(x=w178, y="Error_Stop") -> (0:w232:bool)
    n267 = Greater?(x=w188, y="Error_Stop") -> (0:w242:bool)
    n268 = Greater?(x=w180, y="Error_Stop") -> (0:w234:bool)
    n269 = Build Array(w144, w119, w143, w120) -> (w122:bool[][])
    n270 = case shown="True" w240 {
      tunnel: w185 -> [_ w528]
      tunnel: w69 -> [_ w526]
      tunnel: [w521 w523] -> w239
      tunnel: w226 -> [w521 _]
      tunnel: "Inc/Dec 2" -> [_ w522]
      frame False {
      }
      frame True {
        n271 = Greater Than 0?(x=w528) -> (x > 0?=w527:bool)
        n272 = Add(x=w522, y=w526) -> (x+y=w524:dbl)
        n273 = Subtract(x=w526, y=w522) -> (x-y=w525:dbl)
        n274 = Select(t=w524, s=w527, f=w525) -> (s? t:f=w523:dbl)
      }
    }
    n275 = case shown="True" w238 {
      tunnel: w183 -> [_ w520]
      tunnel: w70 -> [_ w518]
      tunnel: [w513 w515] -> w237
      tunnel: w227 -> [w513 _]
      tunnel: "Inc/Dec 2" -> [_ w514]
      frame False {
      }
      frame True {
        n276 = Greater Than 0?(x=w520) -> (x > 0?=w519:bool)
        n277 = Add(x=w514, y=w518) -> (x+y=w516:dbl)
        n278 = Subtract(x=w518, y=w514) -> (x-y=w517:dbl)
        n279 = Select(t=w516, s=w519, f=w517) -> (s? t:f=w515:dbl)
      }
    }
    n280 = case shown="True" w236 {
      tunnel: w181 -> [_ w512]
      tunnel: w71 -> [_ w510]
      tunnel: [w505 w507] -> w235
      tunnel: w228 -> [w505 _]
      tunnel: "Inc/Dec 2" -> [_ w506]
      frame False {
      }
      frame True {
        n281 = Greater Than 0?(x=w512) -> (x > 0?=w511:bool)
        n282 = Add(x=w506, y=w510) -> (x+y=w508:dbl)
        n283 = Subtract(x=w510, y=w506) -> (x-y=w509:dbl)
        n284 = Select(t=w508, s=w511, f=w509) -> (s? t:f=w507:dbl)
      }
    }
    n285 = case shown="True" w232 {
      tunnel: w177 -> [_ w496]
      tunnel: w73 -> [_ w494]
      tunnel: [w489 w491] -> w231
      tunnel: w230 -> [w489 _]
      tunnel: "Inc/Dec 2" -> [_ w490]
      frame False {
      }
      frame True {
        n286 = Greater Than 0?(x=w496) -> (x > 0?=w495:bool)
        n287 = Add(x=w490, y=w494) -> (x+y=w492:dbl)
        n288 = Subtract(x=w494, y=w490) -> (x-y=w493:dbl)
        n289 = Select(t=w492, s=w495, f=w493) -> (s? t:f=w491:dbl)
      }
    }
    n290 = case shown="True" w242 {
      tunnel: w187 -> [_ w536]
      tunnel: w68 -> [_ w534]
      tunnel: [w529 w531] -> w241
      tunnel: w48 -> [w529 _]
      tunnel: "Inc/Dec 2" -> [_ w530]
      frame False {
      }
      frame True {
        n291 = Greater Than 0?(x=w536) -> (x > 0?=w535:bool)
        n292 = Add(x=w530, y=w534) -> (x+y=w532:dbl)
        n293 = Subtract(x=w534, y=w530) -> (x-y=w533:dbl)
        n294 = Select(t=w532, s=w535, f=w533) -> (s? t:f=w531:dbl)
      }
    }
    n295 = case shown="True" w234 {
      tunnel: w179 -> [_ w504]
      tunnel: w72 -> [_ w502]
      tunnel: [w497 w499] -> w233
      tunnel: w229 -> [w497 _]
      tunnel: "Inc/Dec 2" -> [_ w498]
      frame False {
      }
      frame True {
        n296 = Greater Than 0?(x=w504) -> (x > 0?=w503:bool)
        n297 = Add(x=w498, y=w502) -> (x+y=w500:dbl)
        n298 = Subtract(x=w502, y=w498) -> (x-y=w501:dbl)
        n299 = Select(t=w500, s=w503, f=w501) -> (s? t:f=w499:dbl)
      }
    }
    n300 = Reshape Array(w122, 32 ("dimension size")) -> ()  [unwired: 1 out]
    n301 = feedback-in #9(w239) -> ()
    n302 = feedback-in #10(w237) -> ()
    n303 = feedback-in #11(w235) -> ()
    n304 = feedback-in #12(w231) -> ()
    n305 = feedback-in #13(w241) -> ()
    n306 = feedback-in #14(w233) -> ()
    n307 = Build Array(w68, w69, w70, w71) -> ()  [unwired: 1 out]
    n308 = call "Convert to Dynamic Data"("Array"=w55) -> ()  [unwired: 3 in, 1 out]
  }
  n309 = call <vilib>:"DAQmx Stop Task.vi"("task/channels in"=w23, "error in"=w24) -> ("task out"=w29:refnum<k21>, "error out"=w28:errorcluster)  [unwired: 12 in]
  n310 = call <vilib>:"DAQmx Stop Task.vi"("task/channels in"=w13, "error in"=w12) -> ("task out"=w16:refnum<k21>, "error out"=w15:errorcluster)  [unwired: 12 in]
  n311 = call <vilib>:"DAQmx Clear Task.vi"("task in"=w29, "error in"=w28) -> ("error out"=w27:errorcluster)  [unwired: 13 in]
  n312 = call <vilib>:"DAQmx Clear Task.vi"("task in"=w16, "error in"=w15) -> ("error out"=w14:errorcluster)  [unwired: 13 in]
  n313 = call <vilib>:"Simple Error Handler.vi"("error in (no error)"=w27) -> ()  [unwired: 4 in, 5 out]
  n314 = call <vilib>:"Simple Error Handler.vi"("error in (no error)"=w14) -> ()  [unwired: 4 in, 5 out]
  n315 = call <vilib>:"zmq_close.vi"("error in"=w36, "socket"=w35) -> ("error out"=w37:errorcluster)  [unwired: 3 in]
  n316 = call <vilib>:"zmq_ctx_destroy.vi"("error in"=w37, "context in"=w38) -> ("error out"=→"error out":errorcluster)  [unwired: 3 in]
  n317 = call-poly <vilib>:"DAQmx Create Virtual Channel.vi"("physical channels"=tag "cDAQ1Mod7/ao0") -> ("task out"=w10:refnum<k21>, "error out"=w11:errorcluster)  [unwired: 13 in]
  n318 = property class="DAQmx Channel"(reference=w10, error in=w11, "AO.TermCfg"=w8) -> (reference out=w4:refnum<k21>, error out=w3:errorcluster)
  n319 = while {
    tunnel: w4 -> [w619]
    tunnel: w3 -> [w618]
    tunnel: [w617] -> w2
    tunnel: [w616] -> w1
    stop <- "stop" stop-if-true
    n320 = global read "Trimming_Coil_Command.vi" "Cluster"() -> (w609:T3)
    n321 = Unbundle By Name(w609) -> ("TC9_Set_Point"=w597:dbl)  [unwired: 11 out]
    n322 = Multiply(x=w597, y=1.0) -> (x*y=w600:dbl)
    "TC1_Command" <- w600
    n323 = Divide(x="Error_TC9", y=10000.0) -> (x/y=w598:dbl)
    n324 = Divide(x="Inc/Dec", y=10000000.0) -> (x/y=w604:dbl)
    n325 = feedback #15() -> (w596:dbl)  [unwired: 1 in]
    n326 = Subtract(x=w600, y=w596) -> (x-y=w611:dbl)
    n327 = Absolute Value(x=w611) -> (abs(x)=w612:dbl)
    n328 = Greater?(x=w612, y=w598) -> (0:w610:bool)
    n329 = Multiply(x=w596, y=-100.0) -> (x*y=w613:dbl)
    "Sign*10" <- w613
    n330 = case shown="True" w610 {
      tunnel: w611 -> [_ w627]
      tunnel: w596 -> [_ w625]
      tunnel: [w620 w622] -> w607
      tunnel: w600 -> [w620 _]
      tunnel: w604 -> [_ w621]
      frame False {
      }
      frame True {
        n331 = Greater Than 0?(x=w627) -> (x > 0?=w626:bool)
        n332 = Add(x=w621, y=w625) -> (x+y=w623:dbl)
        n333 = Subtract(x=w625, y=w621) -> (x-y=w624:dbl)
        n334 = Select(t=w623, s=w626, f=w624) -> (s? t:f=w622:dbl)
      }
    }
    "Numeric" <- w607
    n335 = call-poly <vilib>:"DAQmx Write.vi"("task/channels in"=w619, "data"=w613, "error in"=w618) -> ("task out"=w617:refnum<k21>, "error out"=w616:errorcluster)  [unwired: 10 in, 1 out]
    n336 = Multiply(x=w607, y=1.0 ("x")) -> (x*y=→"Waveform Chart":dbl)
    n337 = feedback-in #15(w607) -> ()
  }
  n338 = call <vilib>:"DAQmx Stop Task.vi"("task/channels in"=w2, "error in"=w1) -> ("task out"=w7:refnum<k21>, "error out"=w6:errorcluster)  [unwired: 12 in]
  n339 = call <vilib>:"DAQmx Clear Task.vi"("task in"=w7, "error in"=w6) -> ("error out"=w5:errorcluster)  [unwired: 13 in]
  n340 = call <vilib>:"Simple Error Handler.vi"("error in (no error)"=w5) -> ()  [unwired: 4 in, 5 out]
